vi "onDestroy.vi"(8 "error in (no error)":errorcluster, 11 "Server in":refnum<class "Server.lvclass">) -> (0 "error out":errorcluster, 3 "Server out":refnum<class "Server.lvclass">)   [LabVIEW 2013, in "MQTT Server.lvlib" / "Server.lvclass"]
uses:
  Server.lvclass
  <vilib>/LabVIEW Open Source Project/MQTT Connection/MQTT_Base/Base Class/MQTT_Base.lvclass
  Server.lvclass/Server.ctl
  StoredSessions/StoredSessions.lvclass
  Subscription/_Subscription.lvclass
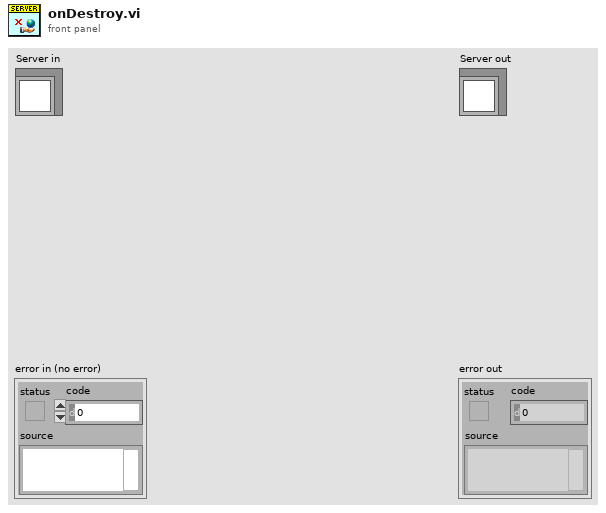
[diagram p1: front panel]
types:
  T1 = typedef "MQTT Server.lvlib/Server.lvclass/Private Events -- cluster.ctl" = cluster{"Inbound Packet":refnum<user-event>, "Inbound Ack":refnum<user-event>}
  T2 = typedef "MQTT Server.lvlib/Server.lvclass/SessionRef -- cluster.ctl" = cluster{"ClientID":string, "SessionMailbox":refnum<queue>}
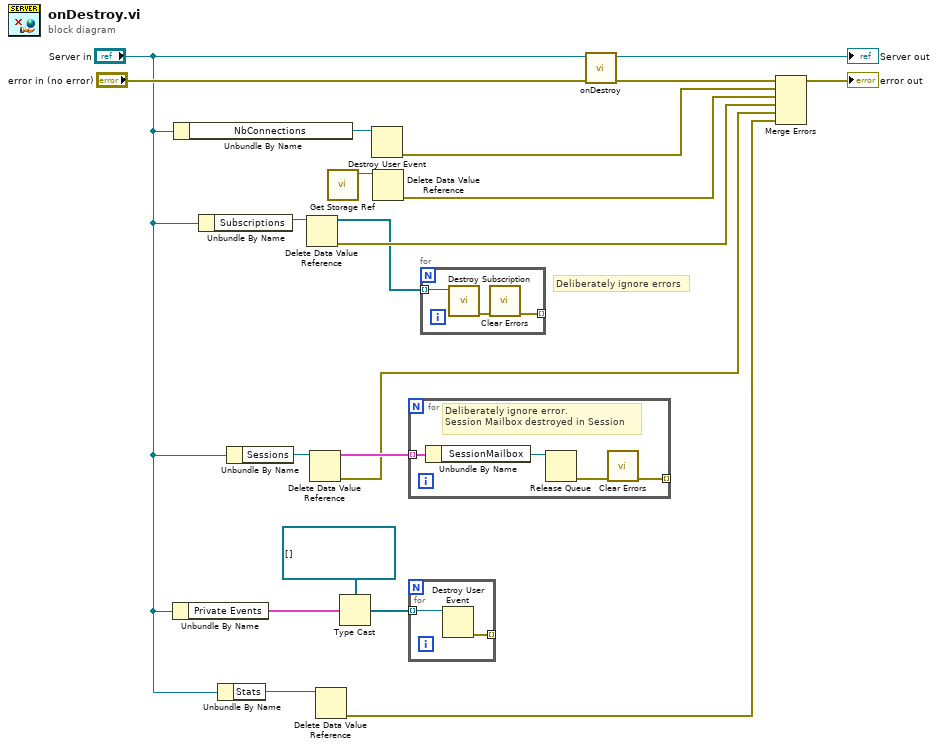
[diagram p0: block diagram]
diagram:
  # "Deliberately ignore errors"
  n1 = Unbundle By Name("Server in") -> ("Private Events"=w4:T1)
  n2 = Unbundle By Name("Server in") -> ("NbConnections"=w17:refnum<user-event>)
  n3 = Unbundle By Name("Server in") -> ("Subscriptions"=w10:refnum<data-value>)
  n4 = Unbundle By Name("Server in") -> ("Stats"=w2:refnum<data-value>)
  n5 = Unbundle By Name("Server in") -> ("Sessions"=w11:refnum<data-value>)
  n6 = Delete Data Value Reference(data value reference=w10) -> (data value=w7:refnum<class "_Subscription.lvclass">[], error out=w9:errorcluster)  [unwired: 1 in]
  n7 = Delete Data Value Reference(data value reference=w11) -> (data value=w12:T2[], error out=w8:errorcluster)  [unwired: 1 in]
  n8 = Delete Data Value Reference(data value reference=w2) -> (error out=w1:errorcluster)  [unwired: 1 in, 1 out]
  n9 = call "Get Storage Ref.vi"() -> ("Storage"=w19:refnum<data-value>)  [unwired: 11 in]
  n10 = Type Cast(type=refnum<user-event>[] [], x=w4) -> (*(type *) &x=w5:refnum<user-event>[])
  n11 = Destroy User Event(user event=w17) -> (error out=w13:errorcluster)  [unwired: 1 in]
  n12 = Delete Data Value Reference(data value reference=w19) -> (error out=w18:errorcluster)  [unwired: 1 in, 1 out]
  n13 = for {
    tunnel: w12 -> [w24] mode=indexing
    tunnel: [w21] -> _ mode=indexing
    # "Deliberately ignore error.\nSession Mailbox destroyed in Session"
    n14 = Unbundle By Name(w24) -> ("SessionMailbox"=w23:refnum<queue>)
    n15 = Release Queue(queue=w23) -> (error out=w22:errorcluster)  [unwired: 2 in, 2 out]
    n16 = call <vilib>:"Clear Errors.vi"("error in (no error)"=w22) -> ("error out"=w21:errorcluster)  [unwired: 6 in]
  }
  n17 = for {
    tunnel: w5 -> [w26] mode=indexing
    tunnel: [w25] -> _ mode=indexing
    n18 = Destroy User Event(user event=w26) -> (error out=w25:errorcluster)  [unwired: 1 in]
  }
  n19 = for {
    tunnel: w7 -> [w29] mode=indexing
    tunnel: [w27] -> _ mode=indexing
    n20 = call "Destroy Subscription.vi"("Subscription in"=w29) -> ("error out"=w28:errorcluster)  [unwired: 9 in, 1 out]
    n21 = call <vilib>:"Clear Errors.vi"("error in (no error)"=w28) -> ("error out"=w27:errorcluster)  [unwired: 6 in]
  }
  n22 = call-parent "onDestroy.vi"("error in (no error)"="error in (no error)", "MQTT_Base in"="Server in") -> ("error out"=w15:errorcluster, "MQTT_Base out"=→"Server out":refnum<class "Server.lvclass">)  [unwired: 8 in]
  n23 = Merge Errors(w15, w13, w18, w9, w8, w1) -> (→"error out":errorcluster)
